vi "LoadSingleToneProfile.vi"(6 "Single Tone":T1 {"Phase" step=0.1 format="%.5f"; "Power" min=0.0 max=0.0009998779334127903 step=5e-05 format="%.9f"; "Frequency" min=0.0 max=500000000.0 format="%.7f"}, 7 "模块路径":path, 8 "PF":u8, 9 "sn":u16, 10 "错误输入（无错误）":errorcluster, 11 "会话句柄输入":refnum<k35>) -> (2 "错误输出":errorcluster, 3 "会话句柄输出":refnum<k35>)   [LabVIEW 2018]
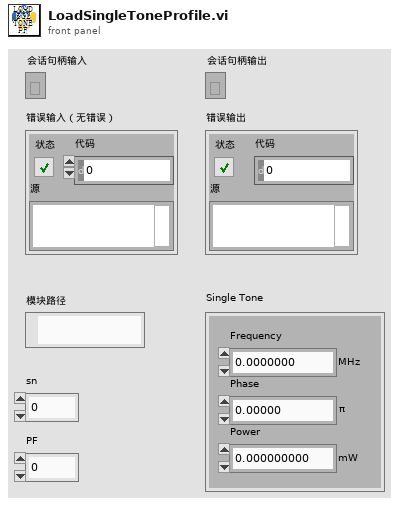
[diagram p1: front panel]
types:
  T1 = cluster{"Frequency":dbl[unit], "Phase":dbl, "Power":dbl[unit]}
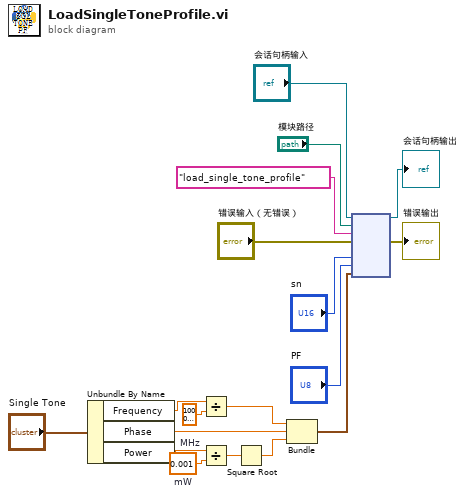
[diagram p0: block diagram]
diagram:
  w9 = dbl[unit] 1000000.0  # MHz
  w8 = dbl[unit] 0.001  # mW
  n1 = Unbundle By Name("Single Tone") -> ("Frequency"=w10:dbl[unit], "Phase"=w4:dbl, "Power"=w7:dbl[unit])
  n2 = Divide(x=w10, y=w9) -> (x/y=w5:dbl)
  n3 = Divide(x=w7, y=w8) -> (x/y=w6:dbl)
  n4 = Square Root(x=w6) -> (sqrt(x)=w3:dbl)
  n5 = Bundle(w5, "Phase"=w4, w3) -> (w2:cluster{dbl, "Phase":dbl, dbl})  [unwired: 1 in]
  n6 = node("会话句柄输入", "模块路径", "load_single_tone_profile", "错误输入（无错误）", "sn", "PF", w2) -> (→"会话句柄输出":refnum<k35>, →"错误输出":errorcluster)  [unwired: 5 in, 2 out]
